vi "FX_Xfer.vi"(8 "error in (no error)":errorcluster, 9 "Data Chars":dbl, 10 "TX":string, 11 "PLC Conn":refnum<visa-resource-name>) -> (1 "error out":errorcluster, 2 "RX":string, 3 "PLC Conn out":refnum<visa-resource-name>)   [LabVIEW 2026]
doc: "Use this template to build a VI to use as a subVI."
panel:
  # "ÕfÃ÷£ºËÍ³ö·â°üKÊÕ»Øª¡£ÏÈ×x 1 Î»Ôª½MÅÐà·Nî£ºSTX ÔÙ×xÙYÁÏ£«\n3£¬ACK¡¢NAK ²»ÓÃÔÙ×x¡£"
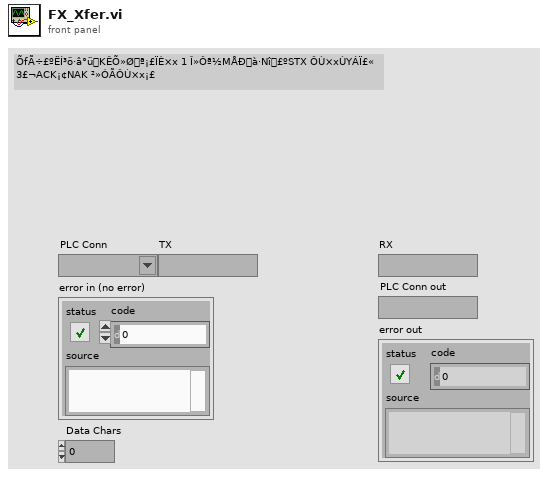
[diagram p1: front panel]
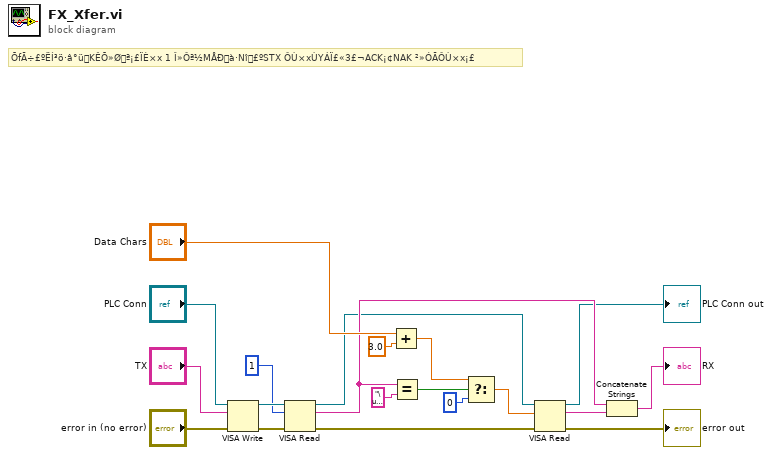
[diagram p0: block diagram]
diagram:
  # "ÕfÃ÷£ºËÍ³ö·â°üKÊÕ»Øª¡£ÏÈ×x 1 Î»Ôª½MÅÐà·Nî£ºSTX ÔÙ×xÙYÁÏ£«3£¬ACK¡¢NAK ²»ÓÃÔÙ×x¡£"
  n1 = VISA Write(VISA resource name="PLC Conn", write buffer="TX", error in (no error)="error in (no error)") -> (VISA resource name out=w19:refnum<visa-resource-name>, error out=w18:errorcluster)  [unwired: 1 out]
  n2 = VISA Read(VISA resource name=w19, byte count=u32 1, error in (no error)=w18) -> (VISA resource name out=w6:refnum<visa-resource-name>, read buffer=w12:string, error out=w5:errorcluster)  [unwired: 1 out]
  n3 = Add(x="Data Chars", y=3.0) -> (x+y=w9:dbl)
  n4 = Equal?(x=w12, y="\u0002") -> (x = y?=w10:bool)
  n5 = Select(t=w9, s=w10, f=0) -> (s? t:f=w7:dbl)
  n6 = VISA Read(VISA resource name=w6, byte count=w7, error in (no error)=w5) -> (VISA resource name out=→"PLC Conn out":refnum<visa-resource-name>, read buffer=w4:string, error out=→"error out":errorcluster)  [unwired: 1 out]
  n7 = Concatenate Strings(w12, w4) -> (→"RX":string)
